vi "RDC-permittivity-Capacitive.vi"(7 "basic data(open, short, water)":T1[](array[typedef]), 11 "Common Format":T1) -> (3 "Common Format 2":T1)   [LabVIEW 2020, in "RDC-Reflection_Data_Computation.lvlib"]
doc: "Computes the permittivity of a Common Format cluster with the Capacative method from the reflections of the basic data (open, short, water) and the water reference permittivity."
uses:
  RDC-Reflection_Data_Computation.lvlib
  Reflector/RFH-common_data_format.ctl
  Reflector/RFH-Reflection_File_Handler.lvlib
panel:
  out "S11 short":cdb[](array[numeric])
  out "S11 open":cdb[](array[numeric])
  out "S11 water":cdb[](array[numeric])
  out "Perm water ref":cdb[](array[numeric])
  out "S11 sample":cdb[](array[numeric])
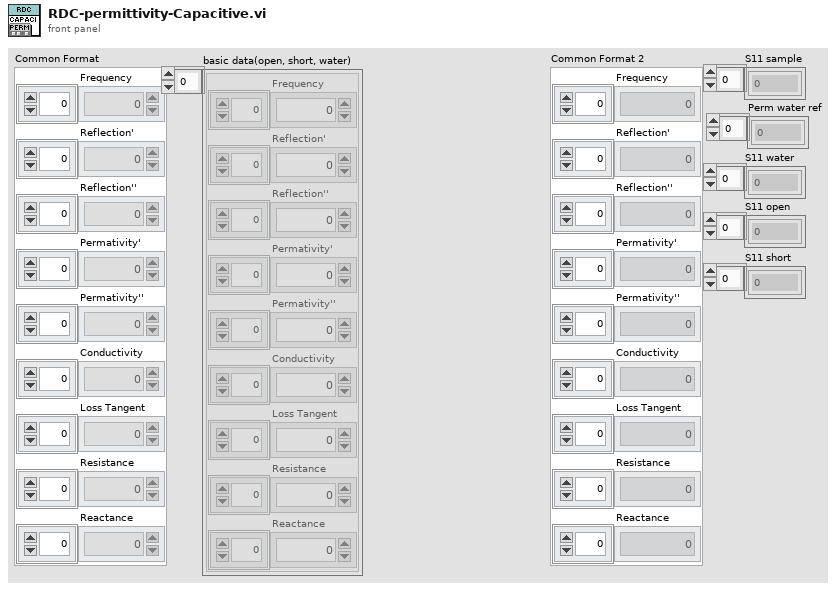
[diagram p1: front panel]
types:
  T1 = typedef "RFH-Reflection_File_Handler.lvlib/RFH-common_data_format.ctl" = cluster{"Frequency":dbl[], "Reflection'":dbl[], "Reflection''":dbl[], "Permativity'":dbl[], "Permativity''":dbl[], "Conductivity":dbl[], "Loss Tangent":dbl[], "Resistance":dbl[], "Reactance":dbl[]}
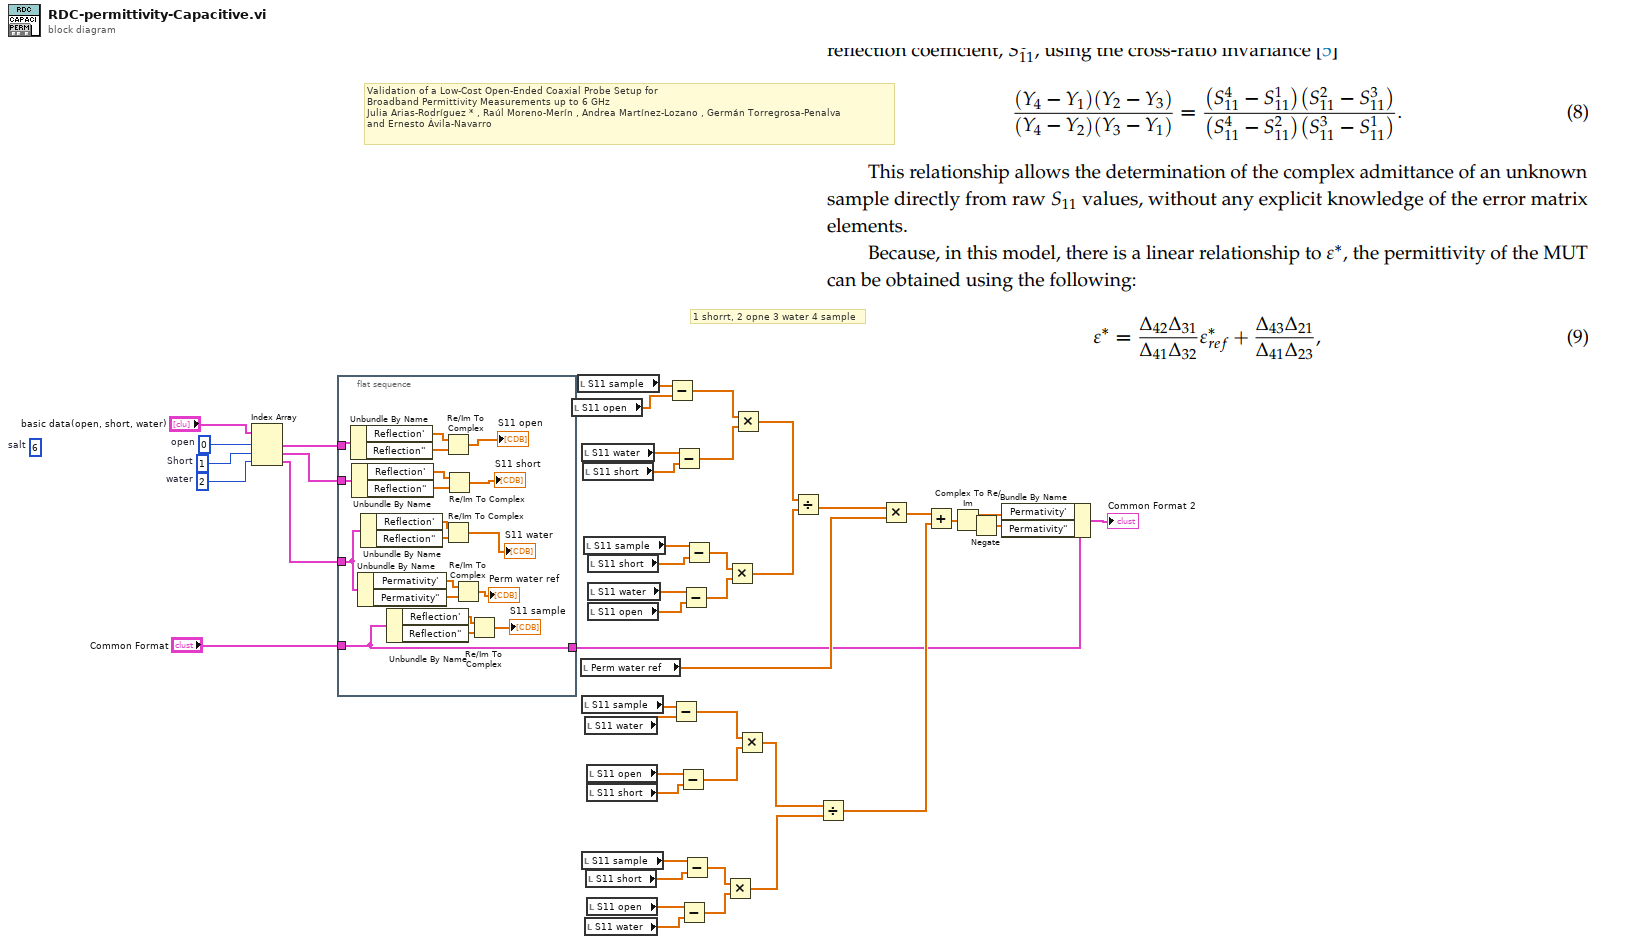
[diagram p0: block diagram]
diagram:
  w2 = 0  # open
  w44 = 2  # water
  w45 = 1  # Short
  (unwired) 6  # salt
  # "1 shorrt, 2 opne 3 water 4 sample"
  # "Validation of a Low-Cost Open-Ended Coaxial Probe Setup for\nBroadband Permittivity Measurements up to 6 GHz\nJulia Arias-Rodríguez * , Raúl Moreno-Merín , Andrea Martínez-Lozano , Germán Torregrosa-Penalva\nand Ernesto Ávila-Navarro"
  n1 = Index Array(array="basic data(open, short, water)", index #1=w2, index #2=w45, index #3=w44) -> (element #1=w7:T1, element #2=w6:T1, element #3=w5:T1)
  n2 = flat-sequence {
    tunnel: w7 -> [w65]
    tunnel: w6 -> [w60]
    tunnel: w5 -> [w51]
    tunnel: [w47] -> w8
    tunnel: "Common Format" -> [w47]
    frame #0 {
      n3 = Unbundle By Name(w65) -> ("Reflection'"=w64:dbl[], "Reflection''"=w63:dbl[])
      n4 = Unbundle By Name(w60) -> ("Reflection'"=w61:dbl[], "Reflection''"=w62:dbl[])
      n5 = Unbundle By Name(w51) -> ("Permativity'"=w53:dbl[], "Permativity''"=w54:dbl[])
      n6 = Unbundle By Name(w51) -> ("Reflection'"=w59:dbl[], "Reflection''"=w58:dbl[])
      n7 = Unbundle By Name(w47) -> ("Reflection'"=w49:dbl[], "Reflection''"=w50:dbl[])
      n8 = Re/Im To Complex(1:w63, 2:w64) -> (0:→"S11 open":cdb[])
      n9 = Re/Im To Complex(1:w58, 2:w59) -> (0:→"S11 water":cdb[])
      n10 = Re/Im To Complex(1:w62, 2:w61) -> (0:→"S11 short":cdb[])
      n11 = Re/Im To Complex(1:w54, 2:w53) -> (0:→"Perm water ref":cdb[])
      n12 = Re/Im To Complex(1:w50, 2:w49) -> (0:→"S11 sample":cdb[])
    }
  }
  n13 = local read "S11 open"() -> (w13:cdb[])
  n14 = local read "S11 sample"() -> (w12:cdb[])
  n15 = local read "Perm water ref"() -> (w38:cdb[])
  n16 = local read "S11 water"() -> (w19:cdb[])
  n17 = local read "S11 sample"() -> (w37:cdb[])
  n18 = local read "S11 sample"() -> (w35:cdb[])
  n19 = local read "S11 short"() -> (w18:cdb[])
  n20 = local read "S11 sample"() -> (w14:cdb[])
  n21 = local read "S11 water"() -> (w36:cdb[])
  n22 = local read "S11 water"() -> (w32:cdb[])
  n23 = local read "S11 short"() -> (w34:cdb[])
  n24 = local read "S11 open"() -> (w30:cdb[])
  n25 = local read "S11 short"() -> (w31:cdb[])
  n26 = local read "S11 open"() -> (w33:cdb[])
  n27 = local read "S11 short"() -> (w15:cdb[])
  n28 = local read "S11 water"() -> (w16:cdb[])
  n29 = local read "S11 open"() -> (w17:cdb[])
  n30 = Subtract(x=w12, y=w13) -> (x-y=w22:cdb[])
  n31 = Subtract(x=w37, y=w36) -> (x-y=w27:cdb[])
  n32 = Subtract(x=w19, y=w18) -> (x-y=w23:cdb[])
  n33 = Subtract(x=w30, y=w31) -> (x-y=w26:cdb[])
  n34 = Subtract(x=w33, y=w32) -> (x-y=w28:cdb[])
  n35 = Subtract(x=w16, y=w17) -> (x-y=w21:cdb[])
  n36 = Subtract(x=w35, y=w34) -> (x-y=w29:cdb[])
  n37 = Subtract(x=w14, y=w15) -> (x-y=w20:cdb[])
  n38 = Multiply(x=w29, y=w28) -> (x*y=w42:cdb[])
  n39 = Multiply(x=w20, y=w21) -> (x*y=w25:cdb[])
  n40 = Multiply(x=w22, y=w23) -> (x*y=w24:cdb[])
  n41 = Multiply(x=w27, y=w26) -> (x*y=w41:cdb[])
  n42 = Divide(x=w24, y=w25) -> (x/y=w39:cdb[])
  n43 = Divide(x=w41, y=w42) -> (x/y=w43:cdb[])
  n44 = Multiply(x=w39, y=w38) -> (x*y=w40:cdb[])
  n45 = Add(x=w40, y=w43) -> (x+y=w11:cdb[])
  n46 = Complex To Re/Im(x + iy=w11) -> (x=w10:dbl[], y=w9:dbl[])
  n47 = Negate(x=w9) -> (-x=w1:dbl[])
  n48 = Bundle By Name(cluster=w8, "Permativity'"=w10, "Permativity''"=w1) -> (→"Common Format 2":T1)
